vi "Fire User Event - Stop.vi"(8 "error in (no error)":errorcluster, 11 "Stop Event":refnum<user-event>) -> (0 "error out":errorcluster)   [LabVIEW 2021]
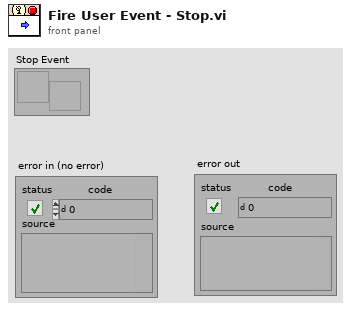
[diagram p1: front panel]
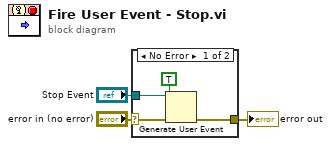
[diagram p0: block diagram]
diagram:
  n1 = case shown="No Error" "error in (no error)" {
    selector: "error in (no error)" -> [w7 w8]
    tunnel: [w6 w8] -> w2
    tunnel: "Stop Event" -> [w5 _]
    frame No Error {
      n2 = Generate User Event(user event=w5, event data cluster=TRUE, error in=w7) -> (error out=w6:errorcluster)  [unwired: 1 in, 1 out]
    }
    frame Error {
    }
  }
  "error out" <- w2
